vi "Start Module.vi"(7 "Panel":refnum<class "Panel.lvclass"> caption="Panel (Window)", 8 "error in (no error)":errorcluster, 11 "Run as Singleton? (F)":bool) -> (0 "error out":errorcluster, 1 "Wait for Event Sync?":bool, 2 "Popup Broadcast Events":T1, 3 "Module ID":i32)   [LabVIEW 2018, in "Popup.lvlib"]
doc: "Launches the Module Main.vi.\n_____\nBased on Delacor QMH Project Template 3.1.0.34."
uses:
  Popup.lvlib
  Broadcast Events--cluster.ctl
  Did Init Argument--cluster.ctl
  Status Updated Argument--cluster.ctl
  Error Reported Argument--cluster.ctl
  Stop Argument--cluster.ctl
  Get Module Execution Status Argument--cluster.ctl
  <vilib>/MGI/Panel Manager/Panel/Panel/Panel.lvclass
  Module Running State--enum.ctl
  <vilib>/Delacor/Delacor QMH/Libraries/Cloneable Module Admin_class/Delacor_lib_QMH_Cloneable Module Admin.lvclass
  C:/Program Files (x86)/National Instruments/LabVIEW 2018/vi.lib/Delacor/Delacor QMH/Libraries/Module Admin_class/Delacor_lib_QMH_Module Admin.lvclass
  <vilib>/Delacor/Delacor QMH/Libraries/Cloneable Module Admin_class/Delacor_lib_QMH_Cloneable Module Admin.lvclass/Delacor_lib_QMH_Cloneable Module Admin.ctl
  <vilib>/Delacor/Delacor QMH/Libraries/Module Admin_class/Delacor_lib_QMH_Module Admin.lvclass/Delacor_lib_QMH_Module Admin.ctl
  <vilib>/Delacor/Delacor QMH/Libraries/Cloneable Module Admin_class/Delacor_lib_QMH_Set Module ID.vi
  <vilib>/Delacor/Delacor QMH/Libraries/Module Admin_class/Delacor_lib_QMH_Set External Launch.vi
  <vilib>/MGI/Panel Manager/Panel/Panel/Window/Window.lvclass
  C:/Program Files (x86)/National Instruments/LabVIEW 2018/vi.lib/MGI/Panel Manager/Panel/Panel/Panel.lvclass
  <vilib>/MGI/Panel Manager/Panel/Panel/Window/Window.vi
  <vilib>/Utility/error.llb/Error Cluster From Error Code.vi
  <vilib>/ErrorRing/Error Ring.xnode
  Clone Registration/Clone Registration.lvlib
  <vilib>/MGI/Panel Manager/Panel/Panel.lvlib
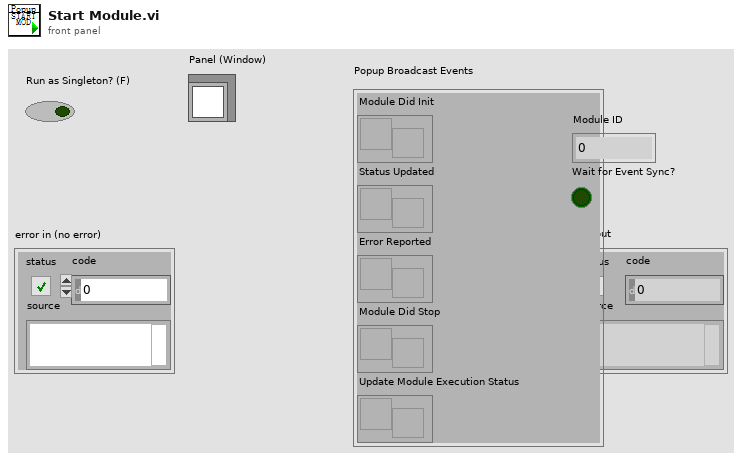
[diagram p1: front panel]
types:
  T1 = typedef "Popup.lvlib/Broadcast Events--cluster.ctl" = cluster{"Module Did Init":refnum<user-event>, "Status Updated":refnum<user-event>, "Error Reported":refnum<user-event>, "Module Did Stop":refnum<user-event>, "Update Module Execution Status":refnum<user-event>}
  T2 = typedef "Popup.lvlib/Module Running State--enum.ctl" = enum16{"Not Running", "Running as Cloneable", "Running as Singleton"}
  T3 = enum32{"Bad", "Idle", "Run top level", "Running"}
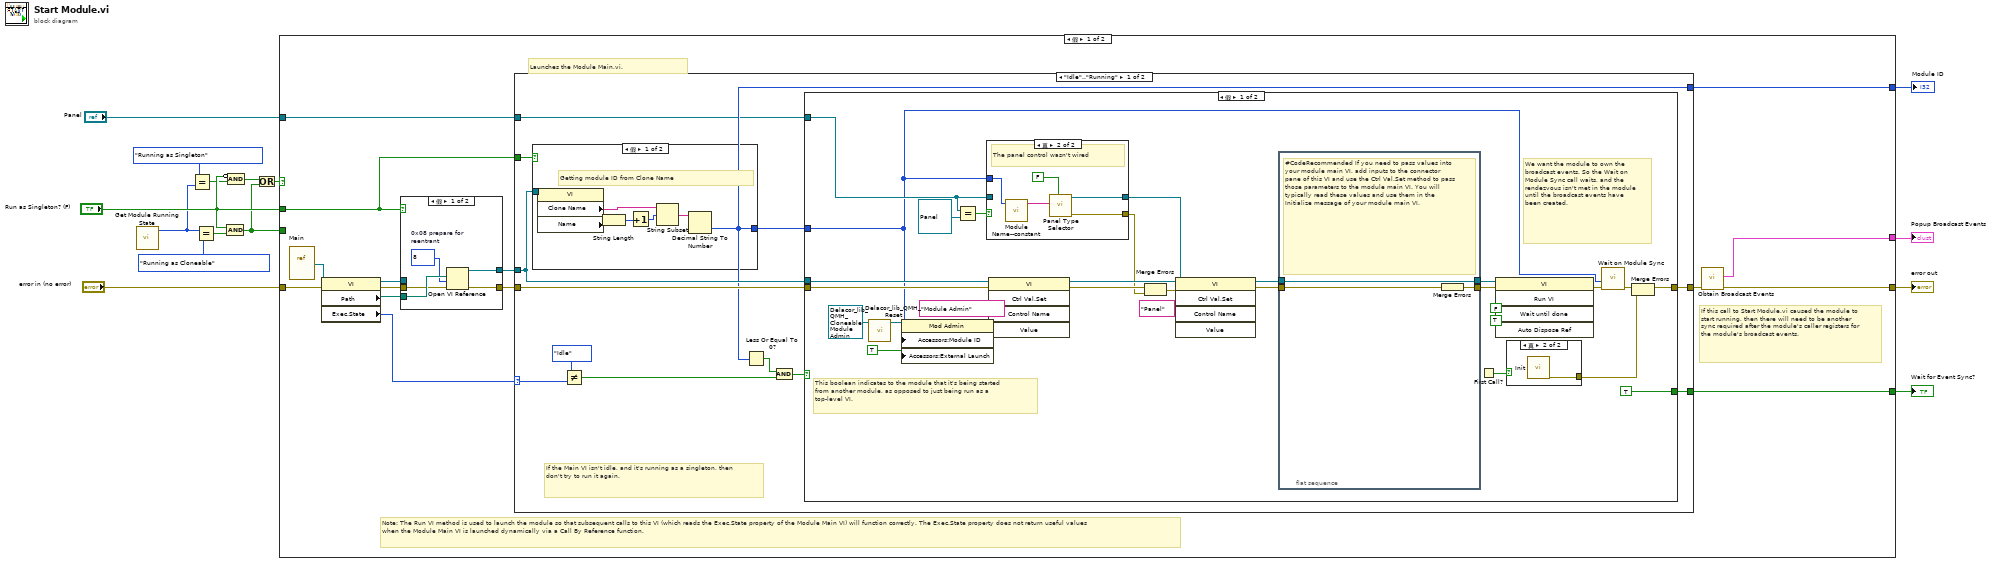
[diagram p0: block diagram]
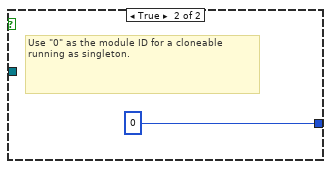
[diagram p3: hidden frame]
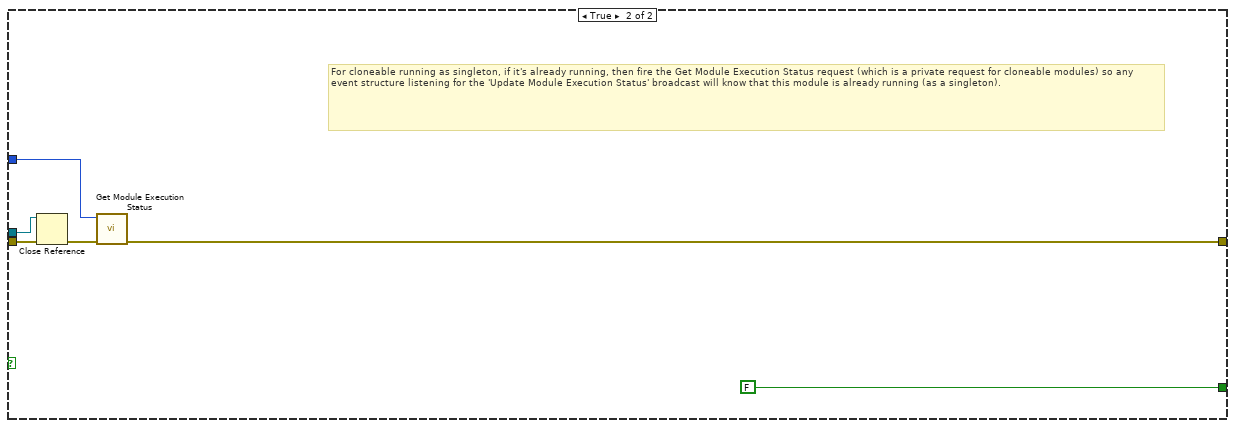
[diagram p6: hidden frame]
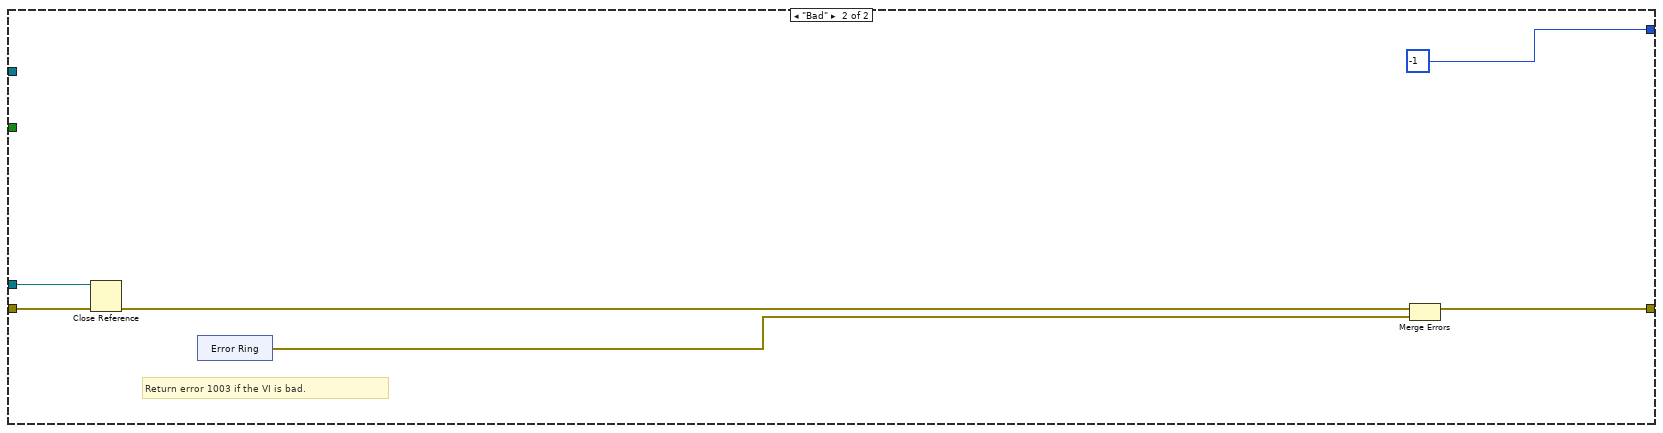
[diagram p7: hidden frame]
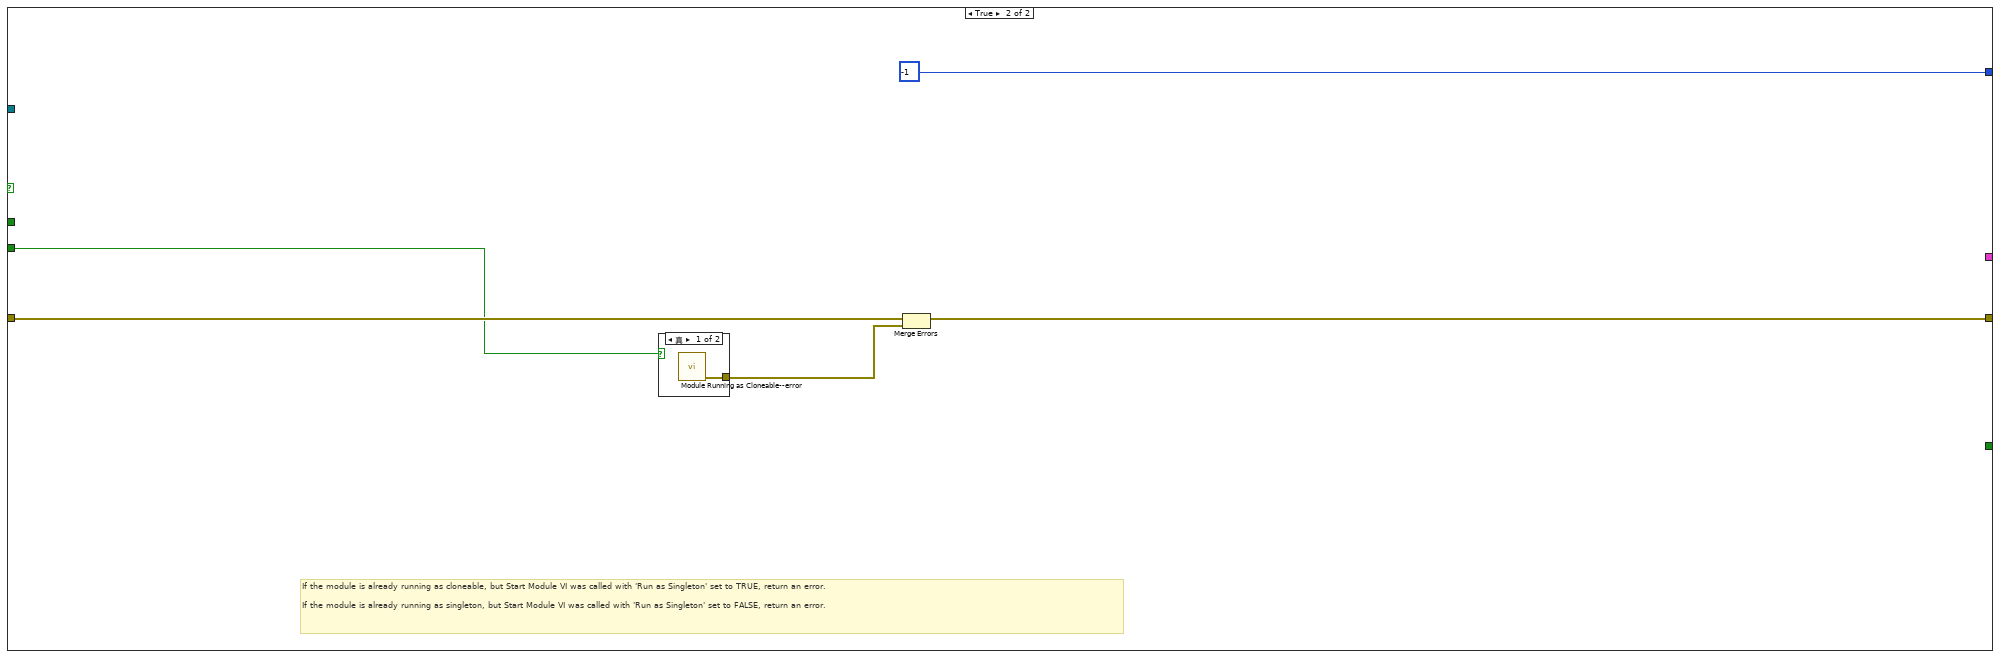
[diagram p8: hidden frame]
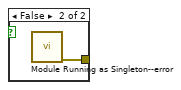
[diagram p9: hidden frame]
diagram:
  n1 = call "Get Module Running State.vi"() -> ("Module Running State"=w4:T2)  [unwired: 11 in]
  n2 = Equal?(x=Module_Running_State--enum."Running as Singleton", y=w4) -> (x = y?=w5:bool)
  n3 = Equal?(x=w4, y=Module_Running_State--enum."Running as Cloneable") -> (x = y?=w9:bool)
  n4 = And(x="Run as Singleton? (F)", y=w9) -> (x .and. y?=w2:bool)
  n5 = Compound Arithmetic op=AND(invert "Run as Singleton? (F)", w5) -> (w7:bool)
  n6 = Or(x=w7, y=w2) -> (x .or. y?=w8:bool)
  n7 = case shown="假" w8 {
    tunnel: "error in (no error)" -> [w30 w117]
    tunnel: [w28 w116] -> w14
    tunnel: [w27 _] -> w13
    tunnel: [w26 _] -> w12
    tunnel: [w22 -1] -> w11
    tunnel: "Run as Singleton? (F)" -> [w18 _]
    tunnel: w2 -> [_ w113]
    tunnel: "Panel" -> [w16 _]
    frame False {
      # "Note: The Run VI method is used to launch the module so that subsequent calls to this VI (which reads the Exec.State property of the Module Main VI) will function correctly. The Exec.State property does not return useful values when the Module Main VI is launched dynamically via a Call By Reference function."
      # "If this call to Start Module.vi caused the module to start running, then there will need to be another sync required after the module's caller registers for the module's broadcast events."
      # "Launches the Module Main.vi."
      n8 = vi-ref "Main.vi"() -> (w21:refnum<vi>)
      n9 = property class="VI"(reference=w21, error in=w30) -> (reference out=w17:refnum<vi>, error out=w24:errorcluster, "Path"=w25:path, "Exec.State"=w19:T3)
      n10 = case shown="假" w18 {
        tunnel: w25 -> [w35 _]
        tunnel: w24 -> [w34 w37]
        tunnel: [w33 w37] -> w23
        tunnel: [w31 w36] -> w20
        tunnel: w17 -> [_ w36]
        frame False {
          w32 = 8  # 0x08 prepare for reentrant
          n11 = Open VI Reference(vi path=w35, options=w32, error in (no error)=w34) -> (vi reference=w31:refnum<vi>, error out=w33:errorcluster)  [unwired: 3 in]
        }
        frame True {
        }
      }
      n12 = case shown="\"Idle\"..\"Running\"" w19 {
        selector: w19 -> [w45 _]
        tunnel: w23 -> [w49 w108]
        tunnel: w20 -> [w47 w107]
        tunnel: [w46 w105] -> w29
        tunnel: [w48 _] -> w26
        tunnel: [w40 -1] -> w22
        tunnel: w18 -> [w39 _]
        tunnel: w16 -> [w38 _]
        frame "Idle".."Running" {
          # "If the Main VI isn't idle, and it's running as a singleton, then don't try to run it again."
          n13 = case shown="假" w39 {
            tunnel: w47 -> [w56 _]
            tunnel: [w50 0] -> w40
            frame False {
              # "Getting module ID from Clone Name"
              n14 = property class="VI"(reference=w56) -> ("Clone Name"=w53:string, "Name"=w52:string)  [unwired: 1 in, 2 out]
              n15 = String Length(string=w52) -> (length=w54:i32)
              n16 = Increment(x=w54) -> (x+1=w55:i32)
              n17 = String Subset ("Getting module ID from Clone Name")(string=w53, offset (0)=w55) -> (substring=w51:string)  [unwired: 1 in]
              n18 = Decimal String To Number(string=w51) -> (number=w50:i32)  [unwired: 2 in, 1 out]
            }
            frame True {
              # "Use \"0\" as the module ID for a cloneable running as singleton."
            }
          }
          n19 = Not Equal?(x=T3."Idle", y=w45) -> (x != y?=w43:bool)
          n20 = Less Or Equal To 0?(x=w40) -> (x <= 0?=w41:bool)
          n21 = And(x=w41, y=w43) -> (x .and. y?=w42:bool)
          n22 = case shown="假" w42 {
            tunnel: w49 -> [w86 w101]
            tunnel: [TRUE FALSE] -> w48
            tunnel: w47 -> [w79 w98]
            tunnel: [w77 w97] -> w46
            tunnel: w40 -> [w58 w100]
            tunnel: w38 -> [w59 _]
            frame False {
              # "We want the module to own the broadcast events. So the Wait on Module Sync call waits, and the rendezvous isn't met in the module until the broadcast events have been created."
              # "This boolean indicates to the module that it's being started from another module, as opposed to just being run as a top-level VI."
              n23 = call-dynamic "Delacor_lib_QMH_Reset.vi"("Mod Admin in"=refnum<class "Delacor_lib_QMH_Cloneable Module Admin.lvclass"> refnum) -> ("Mod Admin out"=w75:refnum<class "Delacor_lib_QMH_Cloneable Module Admin.lvclass">)  [unwired: 9 in, 1 out]
              n24 = property class="Mod Admin"(reference=w75, "Accessors:Module ID"=w58, "Accessors:External Launch"=TRUE) -> (reference out=w74:refnum<class "Delacor_lib_QMH_Cloneable Module Admin.lvclass">)  [unwired: 1 in, 1 out]
              n25 = Equal?(x=w59, y=refnum<class "Panel.lvclass"> refnum) -> (x = y?=w63:bool)
              n26 = case shown="真" w63 {
                tunnel: w59 -> [w87 _]
                tunnel: [w87 w92] -> w62
                tunnel: [_ w90] -> w60
                tunnel: w58 -> [_ w88]
                frame False {
                  # "A panel object was wired in."
                }
                frame True {
                  # "The panel control wasn't wired"
                  n27 = call "Module Name--constant.vi"("Module ID"=w88) -> ("Module Name"=w89:string)  [unwired: 10 in]
                  n28 = call-poly <vilib>:"Panel Type Selector.vi"("Autoshow? (T)"=FALSE, "Default Title"=w89) -> ("error out"=w90:errorcluster, "Window out"=w92:refnum<class "Window.lvclass">)  [unwired: 8 in]
                }
              }
              n29 = invoke class="VI" method="Ctrl Val.Set"(reference=w79, error in=w86, "Control Name"="Module Admin", "Value"=w74) -> (reference out=w68:refnum<vi>, error out=w69:errorcluster)  [unwired: 1 in, 3 out]
              n30 = Merge Errors(w69, w60) -> (w61:errorcluster)
              n31 = invoke class="VI" method="Ctrl Val.Set"(reference=w68, error in=w61, "Control Name"="Panel", "Value"=w62) -> (reference out=w66:refnum<vi>, error out=w65:errorcluster)  [unwired: 1 in, 3 out]
              n32 = flat-sequence {
                tunnel: w66 -> [w95]
                tunnel: [w95] -> w71
                tunnel: w65 -> [w94]
                tunnel: [w93] -> w70
                frame #0 {
                  # "#CodeRecommended If you need to pass values into your module main VI, add inputs to the connector pane of this VI and use the Ctrl Val.Set method to pass those parameters to the module main VI. You will typically read these values and use them in the Initialize message of your module main VI."
                  n33 = Merge Errors(w94) -> (w93:errorcluster)
                }
              }
              n34 = First Call?() -> (First Call?: T/F=w78:bool)
              n35 = invoke class="VI" method="Run VI"(reference=w71, error in=w70, "Wait until done"=FALSE ("Wait Until Done"), "Auto Dispose Ref"=TRUE ("Auto Dispose Reference")) -> (error out=w83:errorcluster)  [unwired: 1 in, 4 out]
              n36 = case shown="真" w78 {
                tunnel: [_ w96] -> w76
                frame False {
                }
                frame True {
                  n37 = call "Init.vi"() -> ("error out"=w96:errorcluster)  [unwired: 8 in, 3 out]
                }
              }
              n38 = call "Wait on Module Sync.vi"("error in (no error)"=w83, "Module ID"=w58) -> ("error out"=w82:errorcluster)  [unwired: 9 in]
              n39 = Merge Errors(w82, w76) -> (w77:errorcluster)
            }
            frame True {
              # "For cloneable running as singleton, if it's already running, then fire the Get Module Execution Status request (which is a private request for cloneable modules) so any event structure listening for the 'Update Module Execution Status' broadcast will know that this module is already running (as a singleton)."
              n40 = Close Reference(reference=w98, error in (no error)=w101) -> (error out=w99:errorcluster)
              n41 = call "Get Module Execution Status.vi"("error in (no error)"=w99, "Module ID"=w100) -> ("error out"=w97:errorcluster)  [unwired: 9 in]
            }
          }
        }
        frame "Bad" {
          # "Return error 1003 if the VI is bad."
          n42 = Close Reference(reference=w107, error in (no error)=w108) -> (error out=w106:errorcluster)
          n43 = xnode "Error Ring"() -> ("错误输出"=w104:errorcluster)
          n44 = Merge Errors(w106, w104) -> (w105:errorcluster)
        }
      }
      n45 = call "Obtain Broadcast Events.vi"("error in (no error)"=w29) -> ("error out"=w28:errorcluster, "Popup Broadcast Events"=w27:T1)  [unwired: 9 in]
    }
    frame True {
      # "If the module is already running as cloneable, but Start Module VI was called with 'Run as Singleton' set to TRUE, return an error.\n\nIf the module is already running as singleton, but Start Module VI was called with 'Run as Singleton' set to FALSE, return an error."
      n46 = case shown="真" w113 {
        tunnel: [w118 w119] -> w114
        frame True {
          n47 = call "Module Running as Cloneable--error.vi"() -> ("error out"=w118:errorcluster)  [unwired: 11 in]
        }
        frame False {
          n48 = call "Module Running as Singleton--error.vi"() -> ("error out"=w119:errorcluster)  [unwired: 11 in]
        }
      }
      n49 = Merge Errors(w117, w114) -> (w116:errorcluster)
    }
  }
  "error out" <- w14
  "Popup Broadcast Events" <- w13
  "Wait for Event Sync?" <- w12
  "Module ID" <- w11
